vi "setVipBuildNumber.vi"() -> ()   [LabVIEW 2015]
uses:
  <vilib>/JKI/VIPM API/command-line/support/VI Package Build Spec Data Cluster_vipm_api.ctl
  <vilib>/JKI/VIPM API/command-line/support/Version Info Cluster_vipm_api.ctl
  <vilib>/Utility/error.llb/DialogType.ctl
  <vilib>/JKI/VIPM API/VIPM API_vipm_api.lvlib
  <vilib>/Wiresmith Technology/G CLI/CLI Class/CLI.lvclass
panel:
  out "Next build number":u32
  out "error out":errorcluster
  out "VI Package Build Spec Data":T1
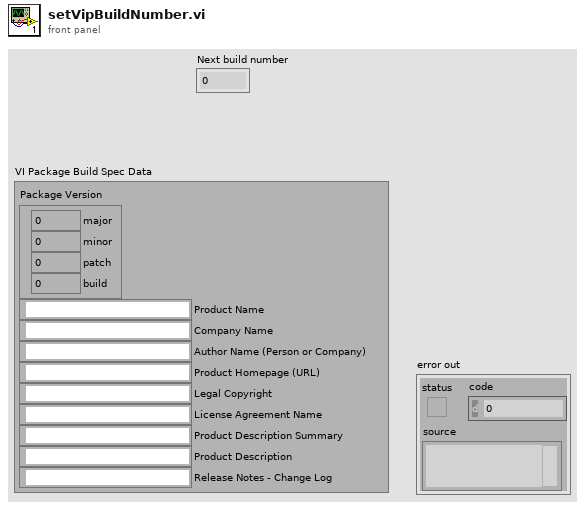
[diagram p1: front panel]
types:
  T1 = typedef "VIPM API_vipm_api.lvlib/VI Package Build Spec Data Cluster_vipm_api.ctl" = cluster{"Package Version":T2, "Product Name":string, "Company Name":string, "Author Name (Person or Company)":string, "Product Homepage (URL)":string, "Legal Copyright":string, "License Agreement Name":string, "Product Description Summary":string, "Product Description":string, "Release Notes - Change Log":string}
  T2 = typedef "VIPM API_vipm_api.lvlib/Version Info Cluster_vipm_api.ctl" = cluster{"major":u32, "minor":u32, "patch":u32, "build":u32}
  T3 = typedef "VIPM API_vipm_api.lvlib/Repository Contents Cluster_vipm_api.ctl" = cluster{"Package Name":string, "Version":string, "Display Name":string, "Release Date":string, "Deprecated":bool}
  T4 = typedef "DialogType.ctl" = u16
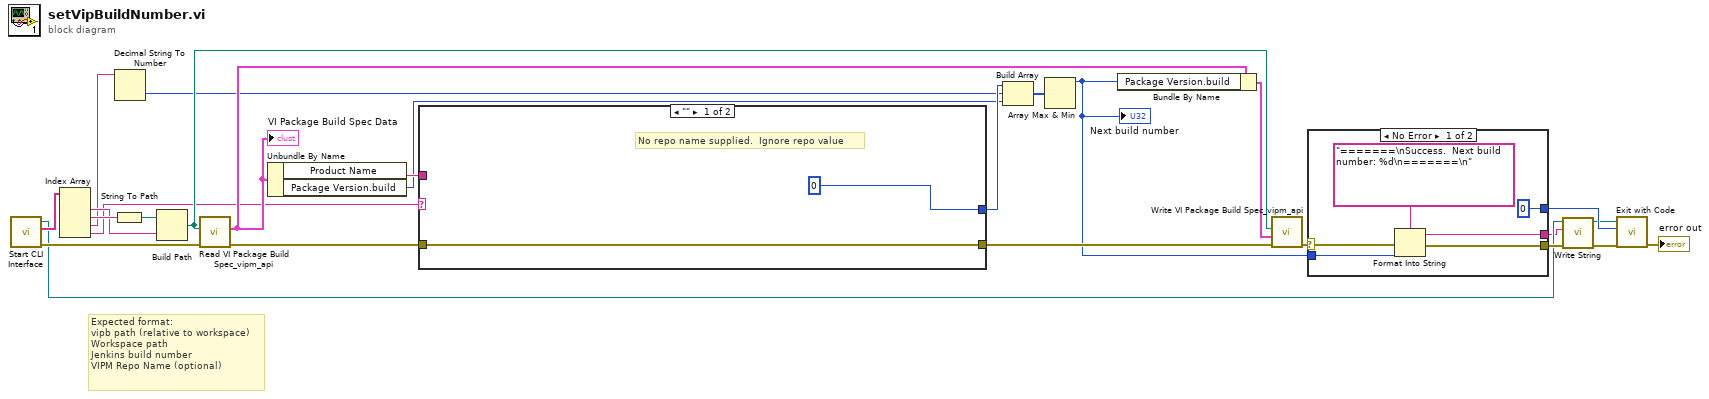
[diagram p0: block diagram]
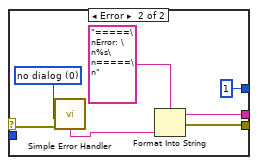
[diagram p2: hidden frame]
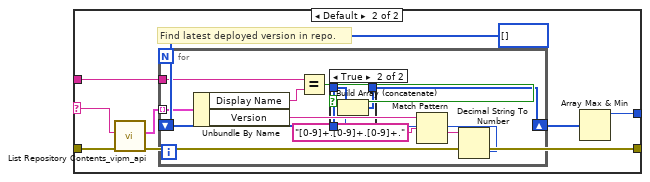
[diagram p3: hidden frame]
diagram:
  # "Expected format:\nvipb path (relative to workspace)\nWorkspace path\nJenkins build number\nVIPM Repo Name (optional)"
  n1 = call <vilib>:"Start CLI Interface.vi"() -> ("error out"=w18:errorcluster, "Custom Parameters"=w16:string[], "CLI out"=w3:refnum<class "CLI.lvclass">)  [unwired: 8 in, 1 out]
  n2 = Index Array(array=w16) -> (element #1=w13:string, element #2=w15:string, element #3=w12:string, element #4=w10:string)  [unwired: 4 in]
  n3 = String To Path(string=w15) -> (path=w14:path)
  n4 = Decimal String To Number(string=w12) -> (number=w11:i32)  [unwired: 2 in, 1 out]
  n5 = Build Path(base path=w14, name or relative path=w13) -> (appended path=w17:path)
  n6 = call <vilib>:"Read VI Package Build Spec_vipm_api.vi"("error in (no error)"=w18, "Path to VIPB File"=w17) -> ("error out"=w23:errorcluster, "VI Package Build Spec Data"=w22:T1)  [unwired: 8 in]
  "VI Package Build Spec Data" <- w22
  n7 = Unbundle By Name(w22) -> ("Product Name"=w21:string, "Package Version.build"=w20:u32)
  n8 = case shown="\"\"" w10 {
    selector: w10 -> [_ w32]
    tunnel: [0 w30] -> w26
    tunnel: [w27 w35] -> w7
    tunnel: w23 -> [w27 w34]
    tunnel: w21 -> [_ w33]
    frame "" {
      # "No repo name supplied.  Ignore repo value"
    }
    frame Default {
      # "Find latest deployed version in repo."
      n9 = call <vilib>:"List Repository Contents_vipm_api.vi"("error in (no error)"=w34, "Repository Name"=w32) -> ("error out"=w35:errorcluster, "Repository Contents []"=w36:T3[])  [unwired: 7 in, 1 out]
      n10 = for {
        tunnel: w36 -> [w46] mode=indexing
        tunnel: w33 -> [w44]
        shift-right: [w37] -> w31
        shift-left: i32[] [] ("Array") -> [w38]
        n11 = Unbundle By Name(w46) -> ("Display Name"=w45:string, "Version"=w41:string)
        n12 = Equal?(x=w44, y=w45) -> (x = y?=w39:bool)
        n13 = Match Pattern(string=w41, regular expression="[0-9]+.[0-9]+.[0-9]+.") -> (after substring=w42:string)  [unwired: 1 in, 3 out]
        n14 = Decimal String To Number(string=w42) -> (number=w40:i32)  [unwired: 2 in, 1 out]
        n15 = case shown="True" w39 {
          tunnel: w38 -> [w47 w49]
          tunnel: w40 -> [_ w48]
          tunnel: [w47 w50] -> w37
          frame False {
          }
          frame True {
            n16 = Build Array (concatenate)(w49, w48) -> (w50:i32[])
          }
        }
      }
      n17 = Array Max & Min(array=w31) -> (max value=w30:i32)  [unwired: 3 out]
    }
  }
  n18 = Build Array(w26, w11, w20) -> (w25:u32[])
  n19 = Array Max & Min(array=w25) -> (max value=w6:u32)  [unwired: 3 out]
  "Next build number" <- w6
  n20 = Bundle By Name(cluster=w22, "Package Version.build"=w6) -> (w24:T1)
  n21 = call <vilib>:"Write VI Package Build Spec_vipm_api.vi"("error in (no error)"=w7, "VI Package Build Spec Data"=w24, "Path to VIPB File"=w17) -> ("error out"=w9:errorcluster)  [unwired: 8 in]
  n22 = case shown="No Error" w9 {
    selector: w9 -> [w54 w60]
    tunnel: [0 ("Exit Code (0)") 1 ("Exit Code (0)")] -> w8
    tunnel: w6 -> [w53 _]
    tunnel: [w52 w62] -> w4
    tunnel: [w51 w61] -> w2
    frame No Error {
      n23 = Format Into String(format string="=======\nSuccess.  Next build number: %d\n=======\n", error in=w54, w53) -> (resulting string=w51:string, error out=w52:errorcluster)  [unwired: 1 in]
    }
    frame Error {
      w57 = T4 0 items=["no dialog", "OK message", "continue or stop message", "OK message + warnings", "continue/stop + warnings"] ("type of dialog (OK msg:1)")
      n24 = call <vilib>:"Simple Error Handler.vi"("type of dialog (OK msg:1)"=w57, "error in (no error)"=w60) -> ("message"=w58:string)  [unwired: 3 in, 4 out]
      n25 = Format Into String(format string="=====\nError: \n%s\n=====\n", w58) -> (resulting string=w61:string, error out=w62:errorcluster)  [unwired: 2 in]
    }
  }
  n26 = call <vilib>:"Write String.vi"("error in (no error)"=w4, "Text to Write"=w2, "CLI in"=w3) -> ("error out"=w5:errorcluster, "CLI out"=w1:refnum<class "CLI.lvclass">)  [unwired: 7 in]
  n27 = call <vilib>:"Exit with Code.vi"("error in (no error)"=w5, "Exit Code (0)"=w8, "CLI in"=w1) -> ("error out"=→"error out":errorcluster)  [unwired: 8 in]
